vi "Read Array Key (Raw).vi"(7 "Section Name":string, 8 "error in (no error)":errorcluster, 10 "Key Name":string, 11 "Config in":T1) -> (0 "error out":errorcluster, 1 "Content":string[](array[string]), 2 "Key Found?":bool, 3 "Config out":T1)   [LabVIEW 2017, in "LabVIEW-Config.lvlib"]
uses:
  LabVIEW-Config.lvlib
  Config.ctl
  LineToken.ctl
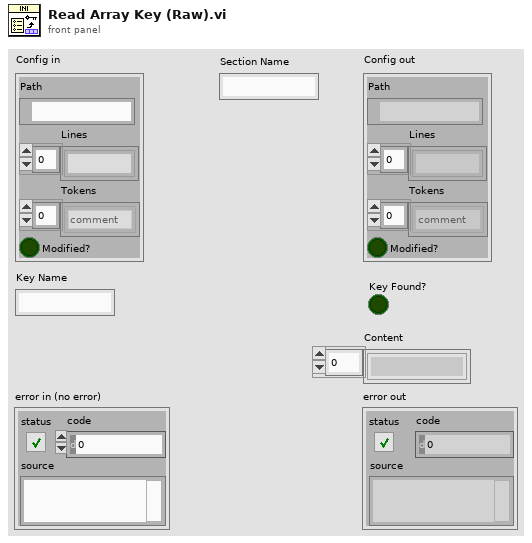
[diagram p1: front panel]
types:
  T1 = typedef "LabVIEW-Config.lvlib/Config.ctl" = cluster{"Path":path, "Lines":string[], "Tokens":T2[], "Modified?":bool}
  T2 = typedef "LabVIEW-Config.lvlib/LineToken.ctl" = enum8{"comment", "section", "key", "more"}
  T3 = typedef "LabVIEW-Config.lvlib/KeyInfo.ctl" = cluster{"Key Indexes":cluster{"Indexes":i32[]}[], "Session Found?":bool, "Key found?":bool, "Session Index":i32}
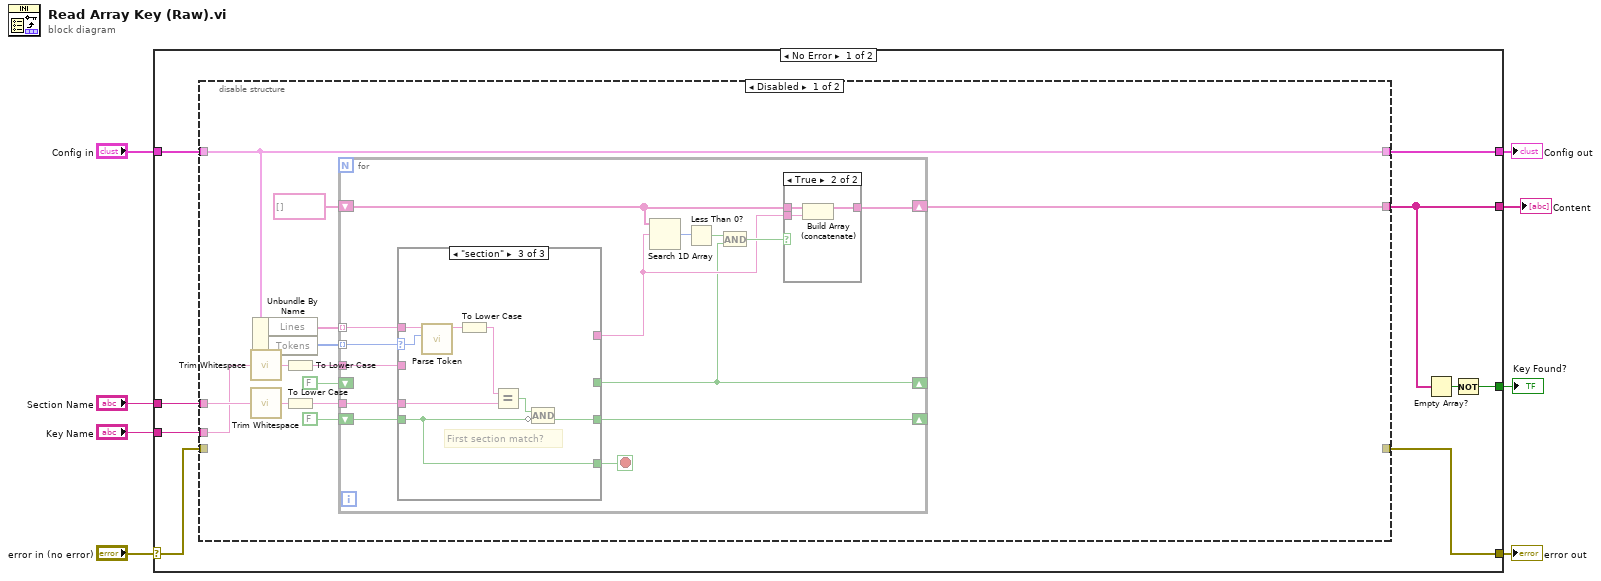
[diagram p0: block diagram]
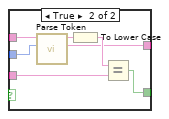
[diagram p5: hidden frame]
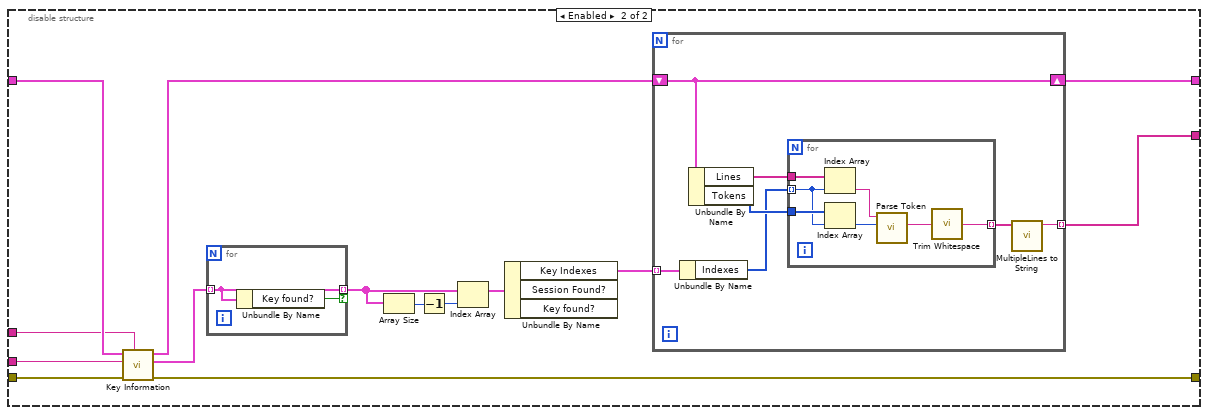
[diagram p6: hidden frame]
diagram:
  n1 = case shown="No Error" "error in (no error)" {
    selector: "error in (no error)" -> [w10 w102]
    tunnel: "Config in" -> [w16 w101]
    tunnel: [w9 w102] -> w7
    tunnel: [w11 w101] -> w5
    tunnel: "Section Name" -> [w17 _]
    tunnel: "Key Name" -> [w15 _]
    tunnel: [w14 _] -> w2
    tunnel: [w12 _] -> w1
    frame No Error {
      n2 = disable-structure shown="Disabled" {
        disable-tunnel: w17 -> [w29 w83]
        disable-tunnel: w16 -> [w18 w84]
        disable-tunnel: w15 -> [w25 w82]
        disable-tunnel: [w21 w71] -> w14
        disable-tunnel: [w18 w72] -> w11
        disable-tunnel: w10 -> [_ w81]
        disable-tunnel: [_ w80] -> w9
        frame Disabled {
          n3 = call <vilib>:"Trim Whitespace.vi"("string"=w25) -> ("trimmed string"=w19:string)  [unwired: 1 in]
          n4 = call <vilib>:"Trim Whitespace.vi"("string"=w29) -> ("trimmed string"=w20:string)  [unwired: 1 in]
          n5 = Unbundle By Name(w18) -> ("Lines"=w30:string[], "Tokens"=w23:T2[])
          n6 = To Lower Case(string=w19) -> (all lower case string=w24:string)
          n7 = To Lower Case(string=w20) -> (all lower case string=w28:string)
          n8 = for {
            tunnel: w23 -> [w44] mode=indexing
            tunnel: w30 -> [w43] mode=indexing
            tunnel: w28 -> [w42]
            shift-right: [w40] -> _
            shift-left: FALSE -> [w41]
            shift-right: [w32] -> _
            shift-left: FALSE -> [_]
            tunnel: w24 -> [w39]
            shift-right: [w35] -> w21
            shift-left: string[] [] -> [w34]
            stop <- w31 stop-if-true
            n9 = case shown="\"section\"" w44 {
              selector: w44 -> [_ w50 w65]
              tunnel: w43 -> [_ w55 w66]
              tunnel: w42 -> [_ _ w70]
              tunnel: [w49 w54 w67] -> w40
              tunnel: w41 -> [w49 w54 w63]
              tunnel: w39 -> [_ w53 _]
              tunnel: [_ w52 _] -> w32
              tunnel: [_ w51 _] -> w33
              tunnel: [_ _ w63] -> w31
              frame "comment", "more" {
              }
              frame "key" {
                n10 = case "Key in Section?" shown="False" w54 {
                  tunnel: w55 -> [_ w59]
                  tunnel: w53 -> [_ w62]
                  tunnel: [_ w60] -> w52
                  tunnel: [_ w56] -> w51
                  tunnel: w50 -> [_ w58]
                  frame False {
                  }
                  frame True {
                    n11 = call "Parse Token.vi"("Token"=w58, "Line"=w59) -> ("Value"=w56:string, "Name"=w57:string)  [unwired: 8 in]
                    n12 = To Lower Case(string=w57) -> (all lower case string=w61:string)
                    n13 = Equal?(x=w61, y=w62) -> (x = y?=w60:bool)
                  }
                }
              }
              frame "section" {
                # "First section match?"
                n14 = call "Parse Token.vi"("Token"=w65, "Line"=w66) -> ("Name"=w64:string)  [unwired: 8 in, 1 out]
                n15 = To Lower Case(string=w64) -> (all lower case string=w69:string)
                n16 = Equal?(x=w69, y=w70) -> (x = y?=w68:bool)
                n17 = Compound Arithmetic op=AND(w68, invert w63) -> (w67:bool)
              }
            }
            n18 = Search 1D Array(1D array=w34, element=w33) -> (index of element=w38:i32)  [unwired: 1 in]
            n19 = Less Than 0?(x=w38) -> (x < 0?=w37:bool)
            n20 = And(x=w37, y=w32) -> (x .and. y?=w36:bool)
            n21 = case shown="True" w36 {
              tunnel: [w45 w48] -> w35
              tunnel: w34 -> [w45 w47]
              tunnel: w33 -> [_ w46]
              frame False {
              }
              frame True {
                n22 = Build Array (concatenate)(w47, w46) -> (w48:string[])
              }
            }
          }
        }
        frame Enabled {
          n23 = call "Key Information.vi"("Section Name"=w83, "error in (no error)"=w81, "Key Name"=w82, "Config in"=w84) -> ("error out"=w80:errorcluster, "Key Information"=w74:T3[], "Config out"=w73:T1)  [unwired: 5 in]
          n24 = for {
            tunnel: w74 -> [w100] mode=indexing
            tunnel: [w100] -> w75 mode=indexing if=w99
            n25 = Unbundle By Name(w100) -> ("Key found?"=w99:bool)
          }
          n26 = Array Size(array=w75) -> (size(s)=w77:i32)
          n27 = Decrement(x=w77) -> (x-1=w76:i32)
          n28 = Index Array(array=w75, index=w76) -> (element=w78:T3)
          n29 = Unbundle By Name(w78) -> ("Key Indexes"=w79:cluster{"Indexes":i32[]}[])  [unwired: 2 out]
          n30 = for {
            tunnel: w79 -> [w88] mode=indexing
            shift-right: [w86] -> w72
            shift-left: w73 -> [w86]
            tunnel: [w85] -> w71 mode=indexing
            n31 = Unbundle By Name(w88) -> ("Indexes"=w87:i32[])
            n32 = Unbundle By Name(w86) -> ("Lines"=w91:string[], "Tokens"=w90:T2[])
            n33 = for {
              tunnel: w91 -> [w98]
              tunnel: w87 -> [w95] mode=indexing
              tunnel: w90 -> [w96]
              tunnel: [w92] -> w89 mode=indexing
              n34 = Index Array(array=w98, index=w95) -> (element=w97:string)
              n35 = Index Array(array=w96, index=w95) -> (element=w94:T2)
              n36 = call "Parse Token.vi"("Token"=w94, "Line"=w97) -> ("Value"=w93:string)  [unwired: 8 in, 1 out]
              n37 = call <vilib>:"Trim Whitespace.vi"("string"=w93) -> ("trimmed string"=w92:string)  [unwired: 1 in]
            }
            n38 = call "MultipleLines to String.vi"("Array"=w89) -> ("String"=w85:string)  [unwired: 10 in]
          }
        }
      }
      n39 = Empty Array?(array=w14) -> (empty?=w13:bool)
      n40 = Not(x=w13) -> (.not. x?=w12:bool)
    }
    frame Error {
    }
  }
  "error out" <- w7
  "Config out" <- w5
  "Content" <- w2
  "Key Found?" <- w1
